vi "BinaryFormatSaveLoop.vi"(7 "Controls ref.":T2, 8 "data error in":errorcluster, 9 "data queue in":refnum<queue>, 10 "control queue in":errorcluster, 11 "control queue in":refnum<queue>) -> (0 "queue error out":errorcluster, 1 "error out":errorcluster, 2 "Quit Binary":bool, 3 "Format":T1=enum."Binary Files")   [LabVIEW 2013]
uses:
  WriterState.ctl
  Signal_Segment.ctl
  ControlDef/ProcessingMode.ctl
  SaveControlsRef.ctl
  ControlDef/Files_Format.ctl
  BinaryHeader.ctl
panel:
  out "Numeric":i32
  out "error out 2":errorcluster
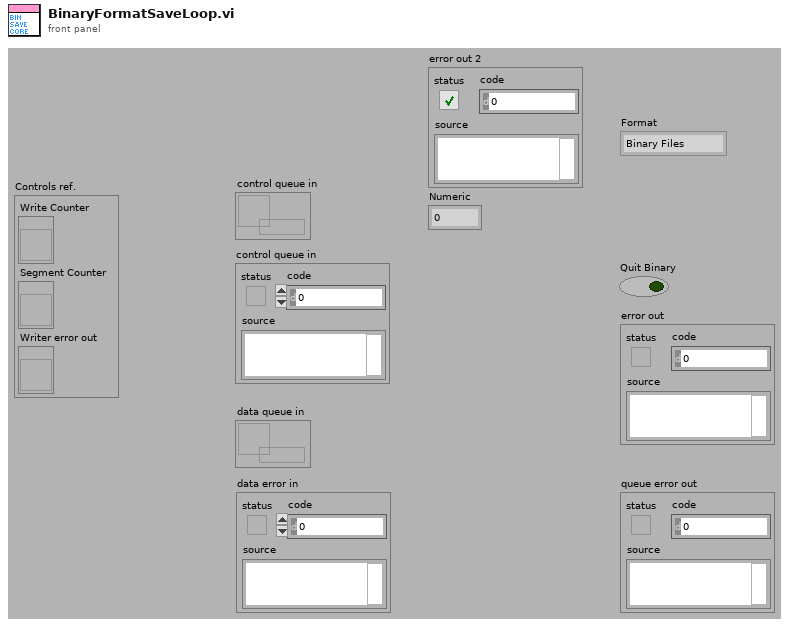
[diagram p1: front panel]
types:
  T1 = typedef "Files_Format.ctl" = enum16{"Text Files", "mzML Files", "Binary Files", "BioMap Files", "imzML Files"}
  T2 = typedef "SaveControlsRef.ctl" = cluster{"Write Counter":refnum<vi>, "Segment Counter":refnum<vi>, "Writer error out":refnum<vi>}
  T3 = enum16{"open", "replace", "create", "open or create", "replace or create", "replace or create with confirmation"}
  T4 = enum16{"big-endian, network order", "native, host order", "little-endian"}
  T5 = typedef "BinaryHeader.ctl" = cluster{"Start Position":dbl[], "StepWidth":dbl[], "Dimension":i32[], "SpecLength":i32}
  T6 = typedef "WriterState.ctl" = cluster{"State":enum16{"Open", "Close", "ChangeFormat", "SetHeader", "QuitProg."}, "Params":variant}
  T7 = enum16{"Open", "Close", "ChangeFormat", "SetHeader", "QuitProg."}
  T8 = typedef "Signal_Segment.ctl" = cluster{"SampleRate":dbl, "TrigDelay":dbl, "SpecLength":dbl, "DAQ_Range":dbl, "Average#":i32, "Position":dbl[], "Spectrum":sgl[], "Calibr.":dbl[], "Pressure":dbl, "Desp_LaserEnergy":dbl, "PI_LaserEnergy":dbl, "Voltages Table":sgl[][], "ProcMode":T9, "Threshold":dbl, "Comment":string, "TickCount":dbl, "Time Stamp":timestamp}
  T9 = typedef "ProcessingMode.ctl" = enum16{"None", "Drop by Threshold", "TDC Simulate", "SetFilter"}
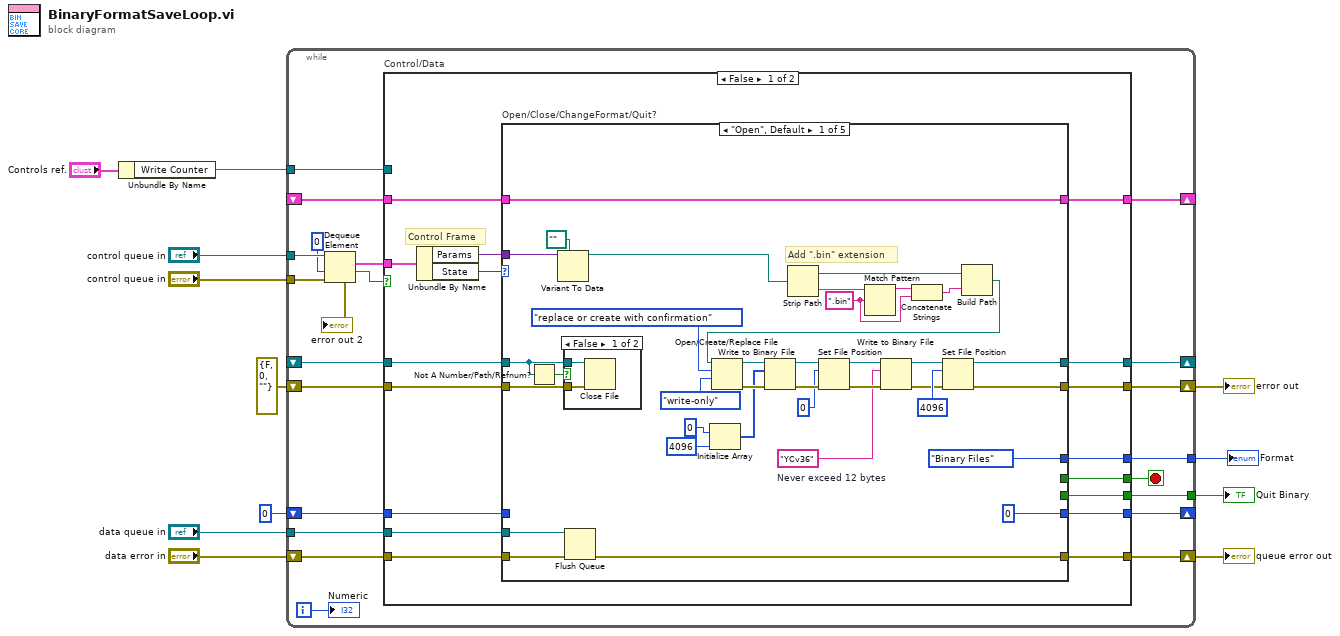
[diagram p0: block diagram]
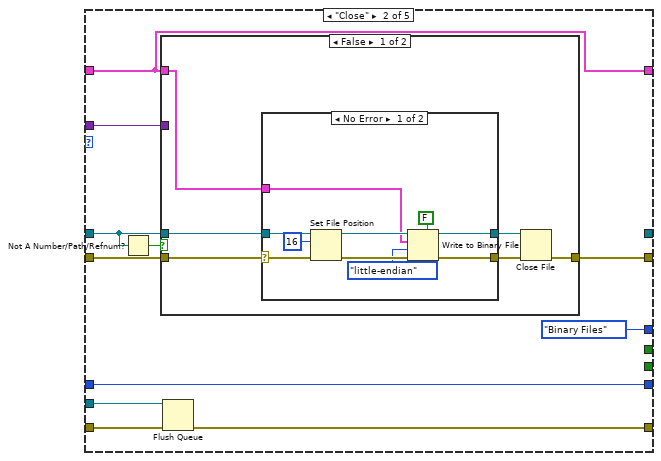
[diagram p3: hidden frame]
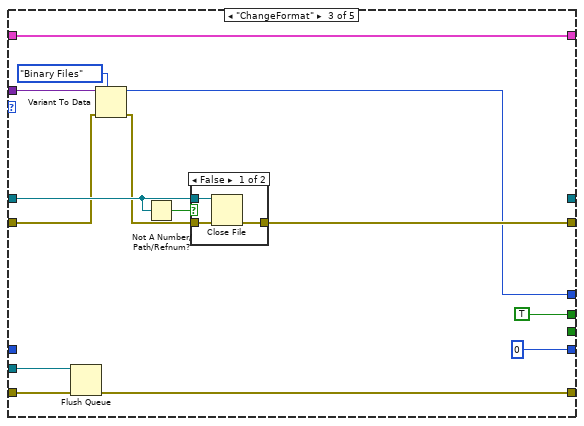
[diagram p6: hidden frame]
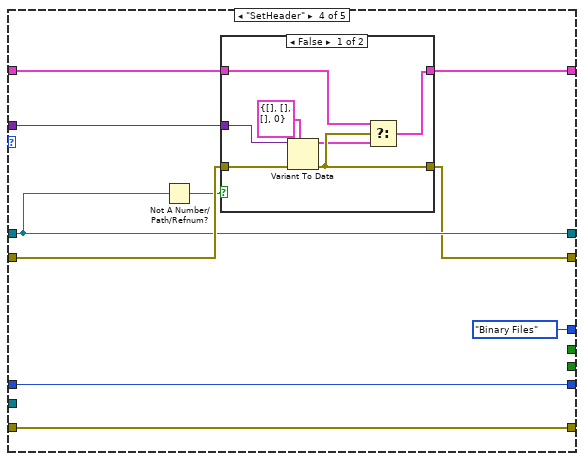
[diagram p8: hidden frame]
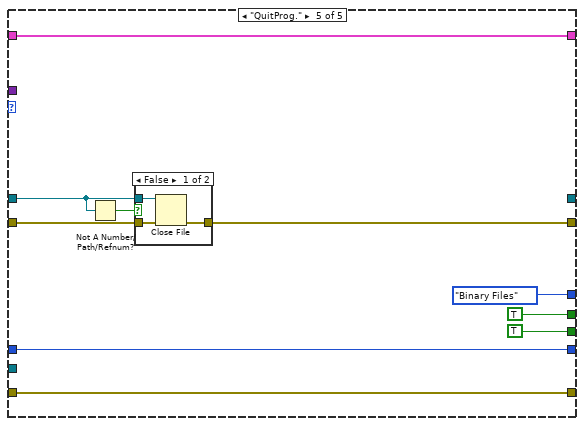
[diagram p10: hidden frame]
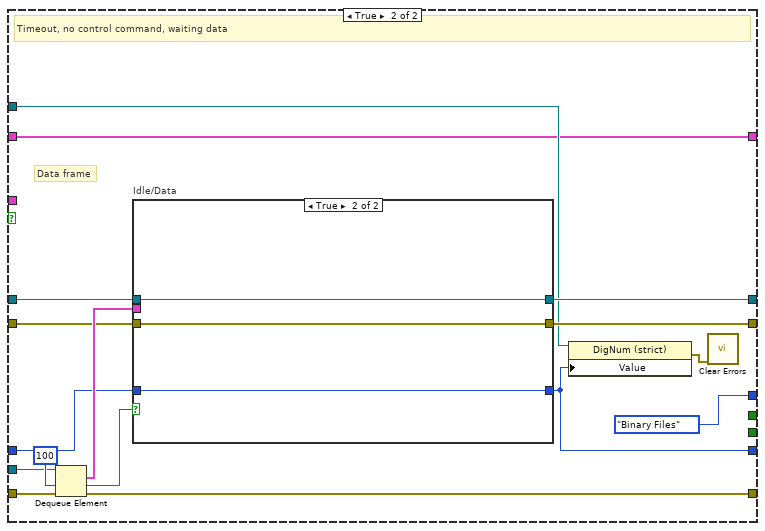
[diagram p12: hidden frame]
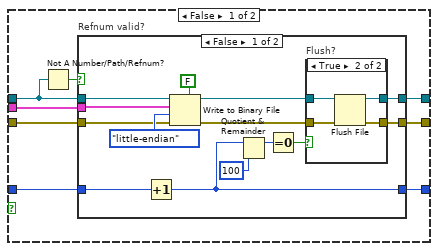
[diagram p13: hidden frame]
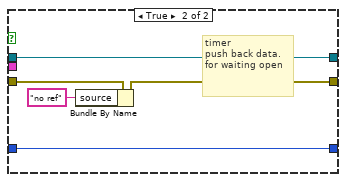
[diagram p15: hidden frame]
diagram:
  n1 = Unbundle By Name("Controls ref.") -> ("Write Counter"=w2:refnum<vi>)
  n2 = while {
    tunnel: [w28] -> w6
    shift-right: [w29] -> _
    shift-left: 0 -> [w34]
    tunnel: "data queue in" -> [w23]
    shift-right: [w32] -> _
    shift-left: _ -> [w33]
    tunnel: "control queue in" -> [w27]
    tunnel: "control queue in" -> [w26]
    tunnel: [w19] -> w1
    shift-right: [w31] -> w5
    shift-left: errorcluster {"status"=FALSE, "code"=0, "source"=""} ("error out") -> [w30]
    tunnel: w2 -> [w17]
    shift-right: [w18] -> w12
    shift-left: "data error in" -> [w22]
    shift-right: [w16] -> _
    shift-left: _ -> [w15]
    i -> [w13]
    stop <- w20 stop-if-true
    n3 = Dequeue Element(queue=w27, timeout in ms (-1)=0, error in (no error)=w26) -> (element=w21:T6, timed out?=w24:bool, error out=→"error out 2":errorcluster)  [unwired: 1 out]
    n4 = case "Control/Data" shown="False" w24 {
      tunnel: w34 -> [w40 w178]
      tunnel: w33 -> [w47 w181]
      tunnel: [w46 w180] -> w32
      tunnel: [w45 w179] -> w31
      tunnel: w30 -> [w48 w182]
      tunnel: [w41 w174] -> w29
      tunnel: [w44 _] -> w28
      tunnel: w23 -> [w38 w185]
      tunnel: w22 -> [w39 w184]
      tunnel: w21 -> [w51 _]
      tunnel: [w43 _] -> w20
      tunnel: [w42 Files_Format."Binary Files" ("Format")] -> w19
      tunnel: [w37 w176] -> w18
      tunnel: w17 -> [_ w175]
      tunnel: [w36 w173] -> w16
      tunnel: w15 -> [w35 w173]
      frame False {
        # "Control Frame"
        n5 = Unbundle By Name(w51) -> ("Params"=w49:variant, "State"=w50:T7)
        n6 = case "Open/Close/ChangeFormat/Quit?" shown="\"Open\", Default" w50 {
          tunnel: w49 -> [w64 w92 w125 w145 _]
          tunnel: w48 -> [w86 w93 w122 w146 w161]
          tunnel: w47 -> [w85 w99 w131 w144 w160]
          tunnel: [w77 _ _ w144 _] -> w46
          tunnel: [w71 w97 w129 w143 w162] -> w45
          tunnel: [_ _ _ _ TRUE] -> w44
          tunnel: [_ _ TRUE _ TRUE] -> w43
          tunnel: [Files_Format."Binary Files" ("Format") Files_Format."Binary Files" ("Format") w124 Files_Format."Binary Files" ("Format") Files_Format."Binary Files" ("Format")] -> w42
          tunnel: [0 w98 0 w147 w164] -> w41
          tunnel: w40 -> [_ w98 _ w147 w164]
          tunnel: w39 -> [w80 w96 w127 w139 w159]
          tunnel: w38 -> [w79 w94 w128 _ _]
          tunnel: [w78 w95 w126 w139 w159] -> w37
          tunnel: [w52 w91 w121 w141 w158] -> w36
          tunnel: w35 -> [w52 w91 w121 w142 w158]
          frame "Open", Default {
            w53 = "YCv36"  # Never exceed 12 bytes
            w70 = ".bin" ("regular expression")
            # "Add \".bin\" extension"
            n7 = Not A Number/Path/Refnum?(number/path/refnum=w85) -> (NaN/Path/Refnum?=w87:bool)
            n8 = Variant To Data(type=path "" ("path"), Variant=w64) -> (data=w62:path)  [unwired: 1 in, 1 out]
            n9 = case shown="False" w87 {
              tunnel: w86 -> [w89 _]
              tunnel: w85 -> [w88 _]
              frame False {
                n10 = Close File(refnum=w88, error in=w89) -> ()  [unwired: 2 out]
              }
              frame True {
              }
            }
            n11 = Flush Queue(queue=w79, error in (no error)=w80) -> (error out=w78:errorcluster)  [unwired: 2 out]
            n12 = Initialize Array(u8 0 ("offset (in bytes) (0)"), 4096 ("dimension size")) -> (w59:u8[])
            n13 = Strip Path(path=w62) -> (stripped path=w66:path, name=w67:string)
            n14 = Match Pattern(string=w67, regular expression=w70) -> (before substring=w69:string)  [unwired: 1 in, 3 out]
            n15 = Concatenate Strings(w69, w70) -> (w68:string)
            n16 = Build Path(base path=w66, name or relative path=w68) -> (appended path=w65:path)
            n17 = Open/Create/Replace File(file path (use dialog)=w65, operation (0:open)=T3."replace or create with confirmation", access (0:read/write)=enum16{"read/write", "read-only", "write-only"}."write-only") -> (refnum out=w76:refnum<file>, error out=w72:errorcluster)  [unwired: 3 in, 1 out]
            n18 = Write to Binary File(file (use dialog)=w76, data=w59, error in=w72) -> (refnum out=w55:refnum<file>, error out=w56:errorcluster)  [unwired: 3 in, 1 out]
            n19 = Set File Position(offset (in bytes) (0)=i64 0, refnum=w55, error in=w56) -> (refnum out=w58:refnum<file>, error out=w57:errorcluster)  [unwired: 1 in]
            n20 = Write to Binary File(file (use dialog)=w58, data=w53, error in=w57) -> (refnum out=w60:refnum<file>, error out=w61:errorcluster)  [unwired: 3 in, 1 out]
            n21 = Set File Position(offset (in bytes) (0)=i64 4096, refnum=w60, error in=w61) -> (refnum out=w77:refnum<file>, error out=w71:errorcluster)  [unwired: 1 in]
          }
          frame "Close" {
            n22 = Not A Number/Path/Refnum?(number/path/refnum=w99) -> (NaN/Path/Refnum?=w100:bool)
            n23 = case shown="False" w100 {
              tunnel: w93 -> [w102 w119]
              tunnel: w99 -> [w105 _]
              tunnel: [w106 w119] -> w97
              tunnel: w92 -> [_ _]
              tunnel: w91 -> [w101 _]
              frame False {
                n24 = case shown="No Error" w102 {
                  selector: w102 -> [w111 w117]
                  tunnel: w105 -> [w116 w118]
                  tunnel: [w114 w118] -> w104
                  tunnel: [w113 w117] -> w103
                  tunnel: w101 -> [w107 _]
                  frame No Error {
                    n25 = Set File Position(offset (in bytes) (0)=i64 16, refnum=w116, error in=w111) -> (refnum out=w115:refnum<file>, error out=w112:errorcluster)  [unwired: 1 in]
                    n26 = Write to Binary File(file (use dialog)=w115, data=w107, error in=w112, 5:FALSE ("prepend array or string size? (T)"), 9:T4."little-endian" ("byte order (0:big-endian, network order)")) -> (refnum out=w114:refnum<file>, error out=w113:errorcluster)  [unwired: 1 in, 1 out]
                  }
                  frame Error {
                  }
                }
                n27 = Close File(refnum=w104, error in=w103) -> (error out=w106:errorcluster)  [unwired: 1 out]
              }
              frame True {
              }
            }
            n28 = Flush Queue(queue=w94, error in (no error)=w96) -> (error out=w95:errorcluster)  [unwired: 2 out]
          }
          frame "ChangeFormat" {
            n29 = Flush Queue(queue=w128, error in (no error)=w127) -> (error out=w126:errorcluster)  [unwired: 2 out]
            n30 = Variant To Data(error in=w122, type=Files_Format."Binary Files" ("Format"), Variant=w125) -> (data=w124:T1, error out=w123:errorcluster)
            n31 = Not A Number/Path/Refnum?(number/path/refnum=w131) -> (NaN/Path/Refnum?=w132:bool)
            n32 = case shown="False" w132 {
              tunnel: w123 -> [w136 w137]
              tunnel: w131 -> [w135 _]
              tunnel: [w134 w137] -> w129
              frame False {
                n33 = Close File(refnum=w135, error in=w136) -> (error out=w134:errorcluster)  [unwired: 1 out]
              }
              frame True {
              }
            }
          }
          frame "SetHeader" {
            n34 = Not A Number/Path/Refnum?(number/path/refnum=w144) -> (NaN/Path/Refnum?=w140:bool)
            n35 = case shown="False" w140 {
              tunnel: w146 -> [w154 w155]
              tunnel: w145 -> [w153 _]
              tunnel: [w151 w155] -> w143
              tunnel: w142 -> [w149 w156]
              tunnel: [w148 w156] -> w141
              frame False {
                n36 = Variant To Data(error in=w154, type=T5 {"Start Position"=[], "StepWidth"=[], "Dimension"=[], "SpecLength"=0} ("output cluster"), Variant=w153) -> (data=w150:T5, error out=w151:errorcluster)
                n37 = Select(t=w149, s=w151, f=w150) -> (s? t:f=w148:T5)
              }
              frame True {
              }
            }
          }
          frame "QuitProg." {
            n38 = Not A Number/Path/Refnum?(number/path/refnum=w160) -> (NaN/Path/Refnum?=w163:bool)
            n39 = case shown="False" w163 {
              tunnel: w161 -> [w169 w170]
              tunnel: w160 -> [w168 _]
              tunnel: [w167 w170] -> w162
              frame False {
                n40 = Close File(refnum=w168, error in=w169) -> (error out=w167:errorcluster)  [unwired: 1 out]
              }
              frame True {
              }
            }
          }
        }
      }
      frame True {
        # "Data frame"
        # "Timeout, no control command, waiting data"
        n41 = Dequeue Element(queue=w185, timeout in ms (-1)=100, error in (no error)=w184) -> (element=w183:T8, timed out?=w177:bool, error out=w176:errorcluster)  [unwired: 1 out]
        n42 = case "Idle/Data" shown="True" w177 {
          tunnel: w183 -> [w194 _]
          tunnel: w182 -> [w193 w221]
          tunnel: w181 -> [w191 w222]
          tunnel: [w188 w222] -> w180
          tunnel: [w187 w221] -> w179
          tunnel: w178 -> [w190 w220]
          tunnel: [w189 w220] -> w174
          frame False {
            n43 = Not A Number/Path/Refnum?(number/path/refnum=w191) -> (NaN/Path/Refnum?=w192:bool)
            n44 = case "Refnum valid?" shown="False" w192 {
              tunnel: [w196 w217] -> w187
              tunnel: [w197 w219] -> w188
              tunnel: w194 -> [w206 _]
              tunnel: w191 -> [w205 w219]
              tunnel: w193 -> [w204 w218]
              tunnel: w190 -> [w203 w215]
              tunnel: [w200 w215] -> w189
              frame False {
                n45 = Increment(x=w203) -> (x+1=w200:i32)
                n46 = Write to Binary File(file (use dialog)=w205, data=w206, error in=w204, 5:FALSE ("prepend array or string size? (T)"), 9:T4."little-endian" ("byte order (0:big-endian, network order)")) -> (refnum out=w199:refnum<file>, error out=w198:errorcluster)  [unwired: 1 in, 1 out]
                n47 = Quotient & Remainder(x=w200, y=100) -> (x-y*floor(x/y)=w202:i32)  [unwired: 1 out]
                n48 = Equal To 0?(x=w202) -> (x = 0?=w201:bool)
                n49 = case "Flush?" shown="True" w201 {
                  tunnel: w199 -> [w210 w214]
                  tunnel: [w210 w213] -> w197
                  tunnel: w198 -> [w209 w212]
                  tunnel: [w209 w211] -> w196
                  frame False {
                  }
                  frame True {
                    n50 = Flush File(refnum=w214, error in=w212) -> (refnum out=w213:refnum<file>, error out=w211:errorcluster)
                  }
                }
              }
              frame True {
                # "timer\npush back data.\nfor waiting open"
                n51 = Bundle By Name(cluster=w218, "source"="no ref") -> (w217:errorcluster)
              }
            }
          }
          frame True {
          }
        }
        n52 = property class="DigNum (strict)"(reference=w175, "Value"=w174) -> (error out=w171:errorcluster)  [unwired: 1 in, 1 out]
        n53 = call <vilib>:"Clear Errors.vi"("error in (no error)"=w171) -> ()  [unwired: 6 in, 1 out]
      }
    }
    "Numeric" <- w13
  }
  "queue error out" <- w12
  "Quit Binary" <- w6
  "error out" <- w5
  "Format" <- w1
